vi "Test A.vi"() -> ()   [LabVIEW 2023, in "LabGRAD.lvlib"]
uses:
  LabGRAD.lvlib
  UiObjects/numeric value control.ctl
  Value/value view.ctl
  UiObjects/string control.ctl
  Value/operation.ctl
  Value/get set ini.ctl
  Value/Value.lvclass
  Value/Value.lvclass/Value.ctl
  Value/_multiply value.vi
  Value/_add float.vi
  Value/_power float.vi
  UiObjects/UiObjects.lvclass
panel:
  out "array view":T1[](array[typedef])
  out "grad":T2
  out "Value 2":T2
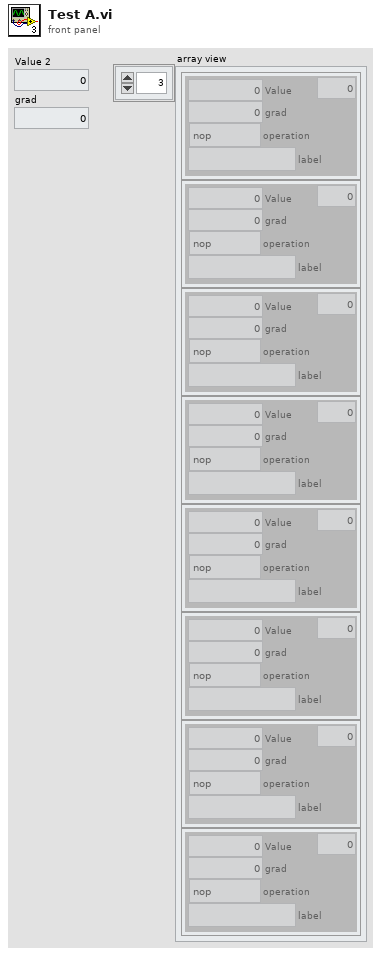
[diagram p1: front panel]
types:
  T1 = typedef "LabGRAD.lvlib/Value.lvclass/value view.ctl" = cluster{"Value":T2, "grad":T2, "label":T3, "operation":T4, "serial":u32}
  T2 = typedef "UiObjects.lvlib/UiObjects.lvclass/numeric value control.ctl" = dbl
  T3 = typedef "UiObjects.lvlib/UiObjects.lvclass/string control.ctl" = string
  T4 = typedef "LabGRAD.lvlib/Value.lvclass/operation.ctl" = enum16{"nop", "add", "subtract", "power", "multiply", "divide", "tanh"}
  T5 = typedef "LabGRAD.lvlib/Value.lvclass/get set ini.ctl" = enum16{"get", "set", "ini"}
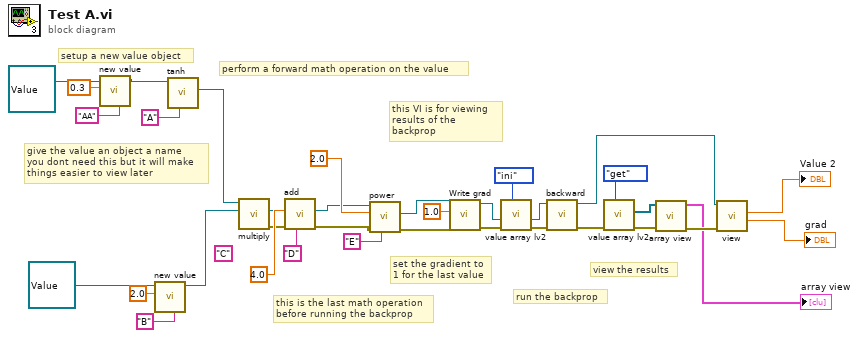
[diagram p0: block diagram]
diagram:
  (unwired) T3 "C" ("label")
  # "view the results"
  # "run the backprop"
  # "this VI is for viewing \nresults of the \nbackprop"
  # "set the gradient to\n1 for the last value"
  # "this is the last math operation\nbefore running the backprop"
  # "perform a forward math operation on the value"
  # "give the value an object a name\nyou dont need this but it will make\nthings easier to view later"
  # "setup a new value object"
  n1 = call "new value.vi"("Label"=T3 "AA", "data"=T2 0.3, "Value in"=refnum<class "Value.lvclass"> refnum ("LabGRAD.lvlib:Value.lvclass")) -> ("Value out"=w9:refnum<class "Value.lvclass">)  [unwired: 7 in, 1 out]
  n2 = call "new value.vi"("Label"=T3 "B", "data"=T2 2.0, "Value in"=refnum<class "Value.lvclass"> refnum ("LabGRAD.lvlib:Value.lvclass")) -> ("Value out"=w4:refnum<class "Value.lvclass">)  [unwired: 7 in, 1 out]
  n3 = call "tanh.vi"("label"=T3 "A", "A"=w9) -> ("C"=w5:refnum<class "Value.lvclass">)  [unwired: 7 in, 2 out]
  n4 = call-poly "multiply.vi"("B"=w4, "A"=w5) -> ("error out"=w7:errorcluster, "C"=w6:refnum<class "Value.lvclass">)  [unwired: 7 in, 1 out]
  n5 = call-poly "add.vi"("label"=T3 "D", "i"=w7, "B"=T2 4.0, "A"=w6) -> ("error out"=w26:errorcluster, "c"=w25:refnum<class "Value.lvclass">)  [unwired: 5 in, 1 out]
  n6 = call-poly "power.vi"("label"=T3 "E", "error in (no error)"=w26, "B"=T2 2.0 ("Value"), "A"=w25) -> ("error out"=w28:errorcluster, "C"=w27:refnum<class "Value.lvclass">)  [unwired: 5 in, 1 out]
  n7 = call "Write grad.vi"("error in (no error)"=w28, "Numeric"=T2 1.0, "Value in"=w27) -> ("error out"=w15:errorcluster, "Value out"=w13:refnum<class "Value.lvclass">)  [unwired: 7 in]
  n8 = call "value array lv2.vi"("Enum"=get_set_ini."ini", "i"=w15, "Value in"=w13) -> (0:"out"=w14:errorcluster, 1:"out"=w12:refnum<class "Value.lvclass">)  [unwired: 5 in, 1 out]
  n9 = call "backward.vi"("i"=w14, "In"=w12) -> ("error out"=w10:errorcluster, "Out"=w16:refnum<class "Value.lvclass">)  [unwired: 8 in]
  n10 = call "value array lv2.vi"("Enum"=get_set_ini."get", "i"=w10) -> ("out"=w18:errorcluster, "array out"=w19:refnum<class "Value.lvclass">[])  [unwired: 6 in, 1 out]
  n11 = call "array view.vi"("i"=w18, "array in"=w19) -> ("o"=w17:errorcluster, "array view"=→"array view":T1[])  [unwired: 8 in]
  n12 = call "view.vi"("error in (no error)"=w17, "Value in"=w16) -> ("grad"=→"grad":T2, "Value"=→"Value 2":T2)  [unwired: 5 in, 3 out]
